vi "DAQmx.Auto Configure.vi"(0 "DAQmx in":refnum<class "DAQmx.lvclass">, 11 "error in (no error)":errorcluster) -> (4 "DAQmx out":refnum<class "DAQmx.lvclass">, 6 "Devices":T9[](array[typedef]), 8 "Configuration.AI":T5 {"input terminal configuration" items=[""=-1, "Differential"=10106, "Pseudodifferential"=12529]; "Coupling" items=[""=0, "AC"=10045, "DC"=10050, "GND"=10066]}, 10 "Configuration.AO":T1 {"output terminal configuration" items=[""=-1, "Differential"=10106, "Pseudodifferential"=12529]}, 15 "error out":errorcluster)   [LabVIEW 2019, in "DAQmx.lvclass"]
uses:
  DAQmx.lvclass
  typedefs/DeviceInfo--Cluster.ctl
  typedefs/DAQ.Config.AI--Cluster--Array.ctl
  typedefs/DAQ.Config.AI--Cluster.ctl
  typedefs/DAQ.Config.AI.Coupling--enum.ctl
  typedefs/DAQ.Config.AI.Range--enum.ctl
  typedefs/DAQ.Config.Device Type--enum.ctl
  typedefs/DAQ.Config.AO--Cluster--Array.ctl
  typedefs/DAQ.Config.AO--Cluster.ctl
  typedefs/DAQ.Config.AO.Range--enum.ctl
  DAQmx.lvclass/DAQmx.ctl
  <resource>/objmgr/daqmx.rc
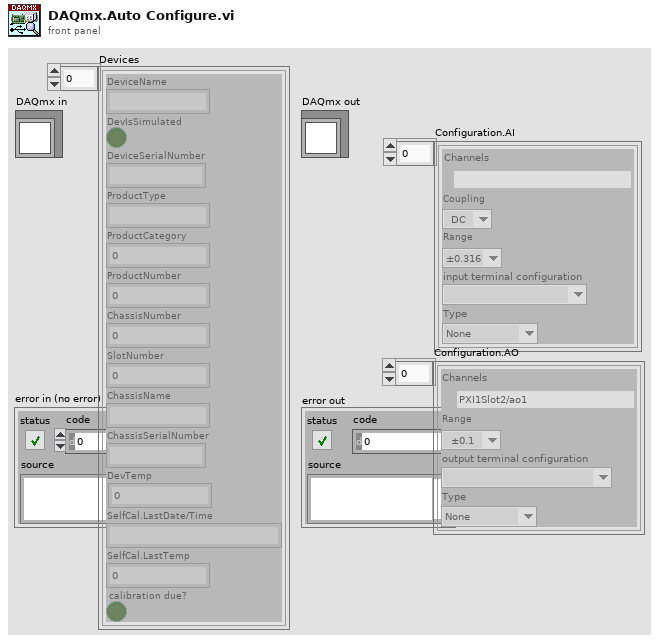
[diagram p1: front panel]
types:
  T1 = typedef "DAQmx.lvclass/DAQ.Config.AO--Cluster--Array.ctl" = T2[]
  T2 = typedef "DAQmx.lvclass/DAQ.Config.AO--Cluster.ctl" = cluster{"Channels":tag, "Range":T3, "output terminal configuration":i32, "Type":T4}
  T3 = typedef "DAQmx.lvclass/DAQ.Config.AO.Range--enum.ctl" = enum16{"±0.1", "±1.0", "±3.5", "±10.0", ""}
  T4 = typedef "DAQmx.lvclass/DAQ.Config.Device Type--enum.ctl" = enum16{"None", "USB-4431", "PXI-446x"}
  T5 = typedef "DAQmx.lvclass/DAQ.Config.AI--Cluster--Array.ctl" = T6[]
  T6 = typedef "DAQmx.lvclass/DAQ.Config.AI--Cluster.ctl" = cluster{"Channels":tag, "Coupling":T7, "Range":T8, "input terminal configuration":i32, "Type":T4}
  T7 = typedef "DAQmx.lvclass/DAQ.Config.AI.Coupling--enum.ctl" = u16
  T8 = typedef "DAQmx.lvclass/DAQ.Config.AI.Range--enum.ctl" = enum16{"±0.316", "±1.00", "±3.16", "±10.0", "±31.6", "±42.4", ""}
  T9 = typedef "DAQmx.lvclass/DeviceInfo--Cluster.ctl" = cluster{"DeviceName":string, "DevIsSimulated":bool, "DeviceSerialNumber":string, "ProductType":string, "ProductCategory":i32, "ProductNumber":u32, "ChassisNumber":u32, "SlotNumber":u32, "ChassisName":string, "ChassisSerialNumber":string, "DevTemp":dbl, "SelfCal.LastDate/Time":string, "SelfCal.LastTemp":dbl, "calibration due?":bool}
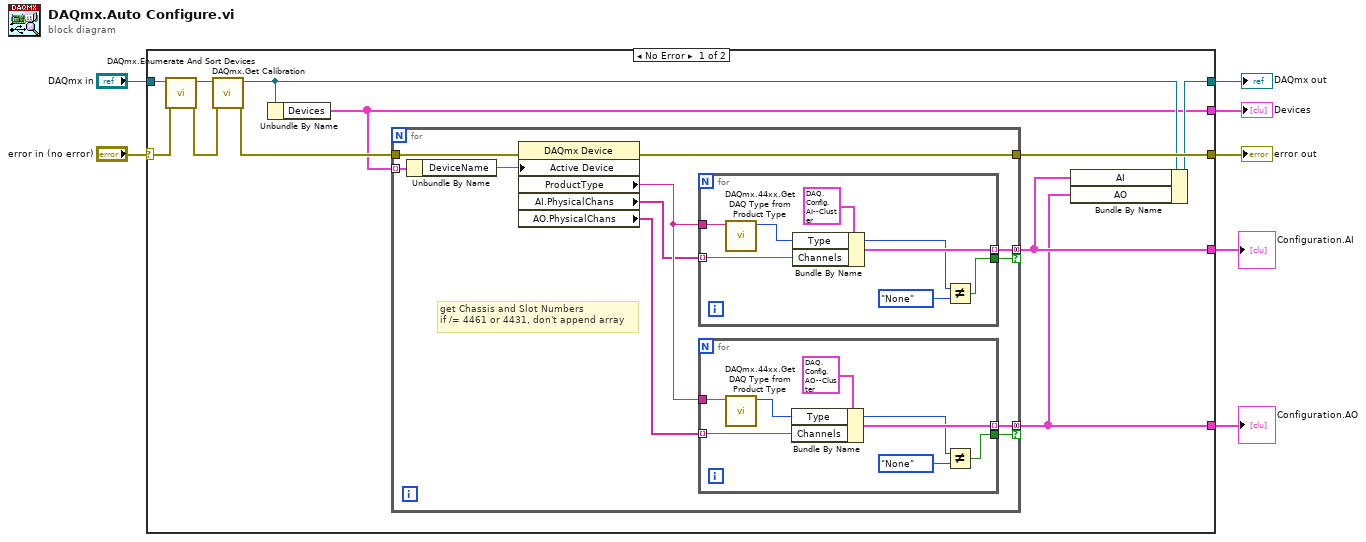
[diagram p0: block diagram]
diagram:
  n1 = case shown="No Error" "error in (no error)" {
    selector: "error in (no error)" -> [w15 w44]
    tunnel: [w18 w44] -> w7
    tunnel: "DAQmx in" -> [w16 w45]
    tunnel: [w17 w45] -> w5
    tunnel: [w8 _] -> w3
    tunnel: [w14 _] -> w2
    tunnel: [w13 _] -> w1
    frame No Error {
      n2 = call "DAQmx.Enumerate And Sort Devices.vi"("error in (no error)"=w15, "DAQmx in"=w16) -> ("error out"=w11:errorcluster, "DAQmx out"=w12:refnum<class "DAQmx.lvclass">)  [unwired: 7 in, 1 out]
      n3 = call "DAQmx.Get Calibration.vi"("error in (no error)"=w11, "DAQmx in"=w12) -> ("error out"=w10:errorcluster, "DAQmx out"=w9:refnum<class "DAQmx.lvclass">)  [unwired: 7 in, 1 out]
      n4 = Unbundle By Name(w9) -> ("Devices"=w8:T9[])
      n5 = for {
        tunnel: [w21] -> w18
        tunnel: [w29] -> w14 mode=concatenating if=w28
        tunnel: w10 -> [w27]
        tunnel: w8 -> [w26] mode=indexing
        tunnel: [w23] -> w13 mode=concatenating if=w22
        # "get Chassis and Slot Numbers\nif /= 4461 or 4431, don't append array"
        n6 = Unbundle By Name(w26) -> ("DeviceName"=w25:string)
        n7 = property class="DAQmx Device"(error in=w27, "Active Device"=w25) -> (error out=w21:errorcluster, "ProductType"=w24:string, "AI.PhysicalChans"=w19:tag[], "AO.PhysicalChans"=w20:tag[])  [unwired: 1 in, 1 out]
        n8 = for {
          tunnel: [w36] -> w29 mode=indexing
          tunnel: w24 -> [w32]
          tunnel: [w31] -> w28
          tunnel: w19 -> [w33] mode=indexing
          n9 = call "DAQmx.44xx.Get DAQ Type from Product Type.vi"("ProductType"=w32) -> ("DAQ Type"=w30:T4)  [unwired: 10 in]
          n10 = Bundle By Name(cluster=T6 {"Channels"="PXI1Slot2/ai0", "Coupling"=10050, "Range"=enum."±0.316", "input terminal configuration"=-1, "Type"=enum."PXI-446x"} ("AI.Config"), "Type"=w30, "Channels"=w33) -> (w36:T6)
          n11 = Not Equal?(x=w30, y=DAQ.Config.Device_Type--enum."None") -> (x != y?=w31:bool)
        }
        n12 = for {
          tunnel: [w39] -> w23 mode=indexing
          tunnel: w24 -> [w43]
          tunnel: [w38] -> w22
          tunnel: w20 -> [w41] mode=indexing
          n13 = call "DAQmx.44xx.Get DAQ Type from Product Type.vi"("ProductType"=w43) -> ("DAQ Type"=w37:T4)  [unwired: 10 in]
          n14 = Bundle By Name(cluster=T2 {"Channels"="PXI1Slot2/ao1", "Range"=enum."±0.1", "output terminal configuration"=-1, "Type"=enum."USB-4431"} ("AO.config"), "Type"=w37, "Channels"=w41) -> (w39:T2)
          n15 = Not Equal?(x=w37, y=DAQ.Config.Device_Type--enum."None") -> (x != y?=w38:bool)
        }
      }
      n16 = Bundle By Name(cluster=w9, "AI"=w14, "AO"=w13) -> (w17:refnum<class "DAQmx.lvclass">)
    }
    frame Error {
    }
  }
  "error out" <- w7
  "DAQmx out" <- w5
  "Devices" <- w3
  "Configuration.AI" <- w2
  "Configuration.AO" <- w1
